vi "ASD Read Candidate.vi"(11 "読み取り配列":string) -> (0 "読み取り長さ":i32, 2 "逆前削減配列マトリクス":string[][](array[string]), 3 "順前削減配列マトリクス":string[][](array[string]))   [LabVIEW 2018]
panel:
  out "順前削減 2":string[](array[string])
  out "逆前削減":string[](array[string])
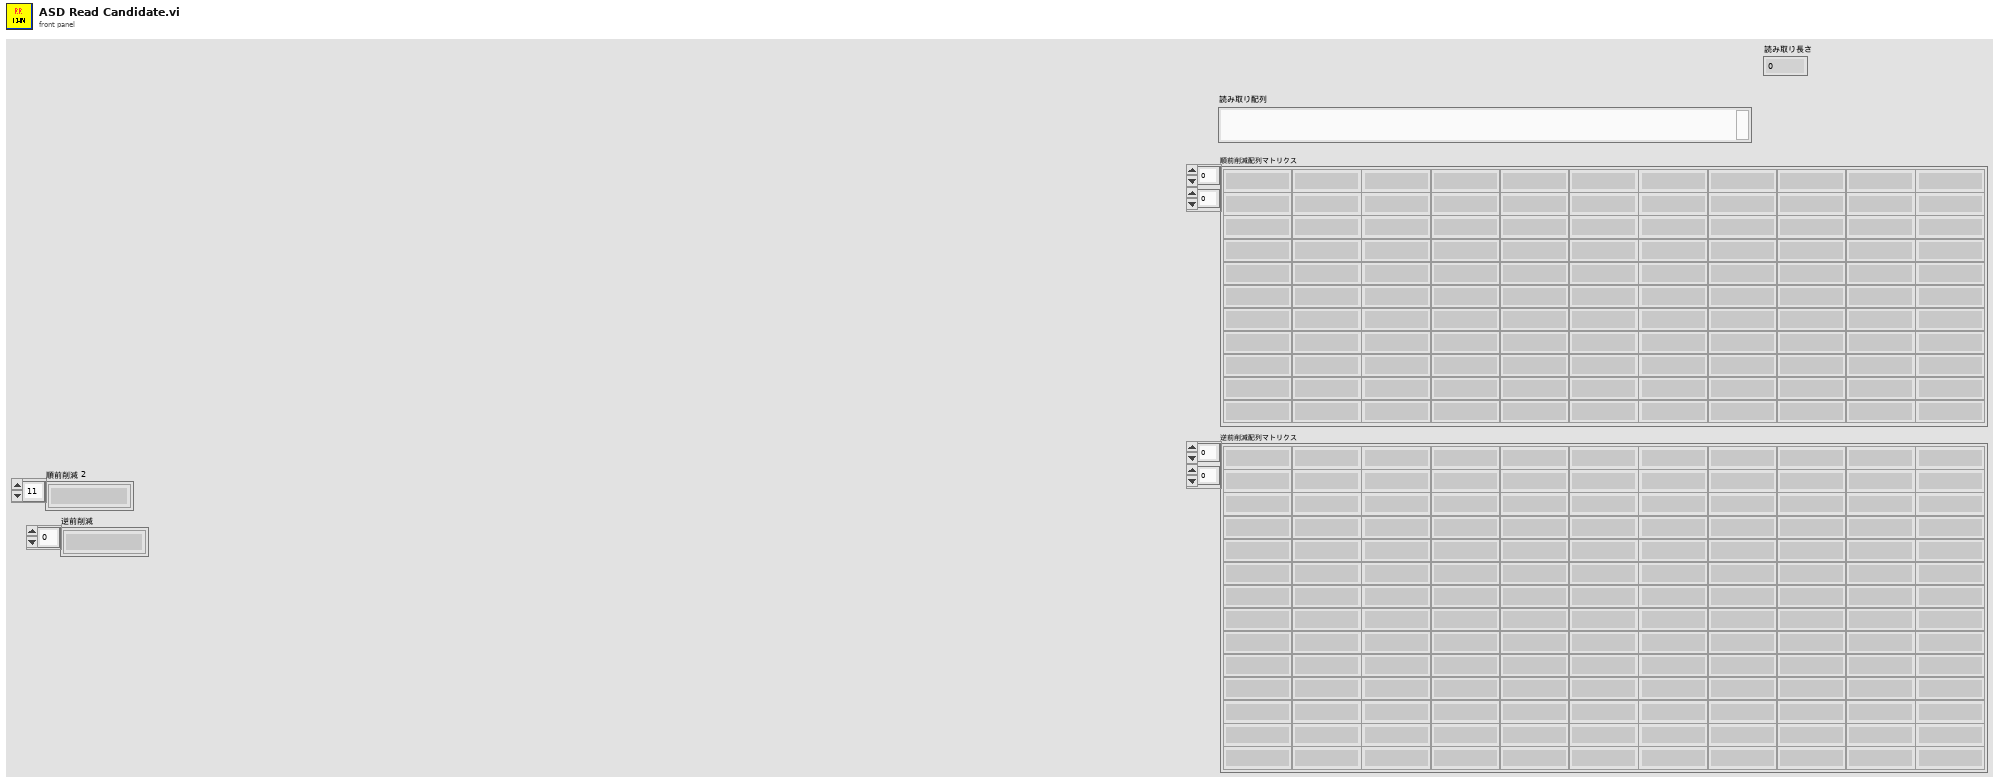
[diagram p1: front panel]
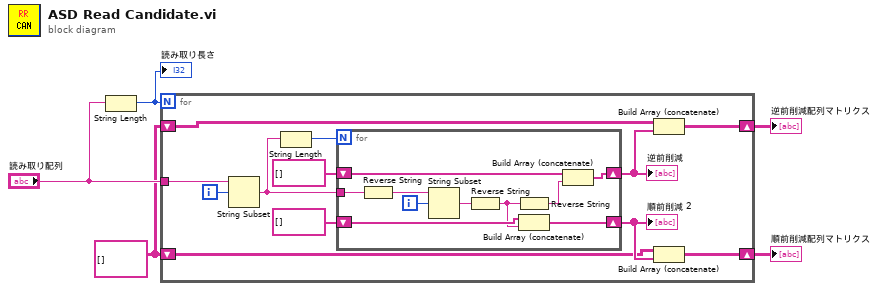
[diagram p0: block diagram]
diagram:
  w3 = string[][] []
  n1 = String Length(string="読み取り配列") -> (length=w4:i32)
  "読み取り長さ" <- w4
  n2 = for {
    N: w4 -> [_]
    tunnel: "読み取り配列" -> [w17]
    shift-right: [w9] -> w2
    shift-left: w3 -> [w10]
    shift-right: [w8] -> w1
    shift-left: w3 -> [w6]
    i -> [w12]
    n3 = String Subset(string=w17, offset (0)=w12) -> (substring=w13:string)  [unwired: 1 in]
    n4 = String Length(string=w13) -> (length=w14:i32)
    n5 = for {
      N: w14 -> [_]
      tunnel: w13 -> [w27]
      shift-right: [w26] -> w11
      shift-left: string[] [] -> [w25]
      shift-right: [w24] -> w7
      shift-left: string[] [] -> [w23]
      i -> [w21]
      n6 = Reverse String(1:w27) -> (0:w19:string)
      n7 = String Subset(string=w19, offset (0)=w21) -> (substring=w22:string)  [unwired: 1 in]
      n8 = Reverse String(1:w22) -> (0:w18:string)
      n9 = Reverse String(1:w18) -> (0:w20:string)
      n10 = Build Array (concatenate)(w25, w18) -> (w26:string[])
      n11 = Build Array (concatenate)(w23, w20) -> (w24:string[])
    }
    "順前削減 2" <- w11
    "逆前削減" <- w7
    n12 = Build Array (concatenate)(w6, w7) -> (w8:string[][])
    n13 = Build Array (concatenate)(w10, w11) -> (w9:string[][])
  }
  "順前削減配列マトリクス" <- w2
  "逆前削減配列マトリクス" <- w1
